vi "report generation.vi"(9 "text":string, 11 "template (empty)":path) -> ()   [LabVIEW 2026]
uses:
  <vilib>/addons/_office/NI_ReportGenerationToolkit.lvlib
  <vilib>/addons/_office/_exclsub.llb/font.ctl
  <vilib>/Utility/NIReport.llb/NI_report.lvclass
  <vilib>/addons/_office/word.llb/Word Easy Table (num).vi
  <vilib>/Utility/NIReport.llb/Report Type.ctl
  <vilib>/Utility/NIReport.llb/NI_ReportGenerationCore.lvlib
panel:
  in  "report type":T1
  in  "error in (no error)":errorcluster
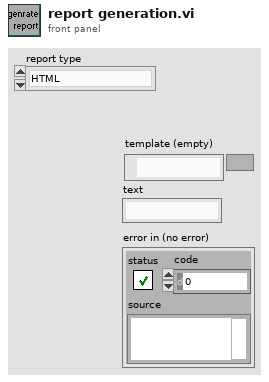
[diagram p1: front panel]
types:
  T1 = typedef "NI_ReportGenerationCore.lvlib/Report Type.ctl" = enum16{"HTML", "Word", "Excel"}
  T2 = typedef "NI_ReportGenerationToolkit.lvlib/font.ctl" = cluster{"font name":string, "font size":dbl, "bold":u16, "italic":u16, "underline":u16, "strike through":u16, "font color":u32}
  T3 = enum16{"maximized", "minimized", "normal", "no change"}
  T4 = enum16{"open", "replace", "create", "open or create", "replace or create", "replace or create with confirmation"}
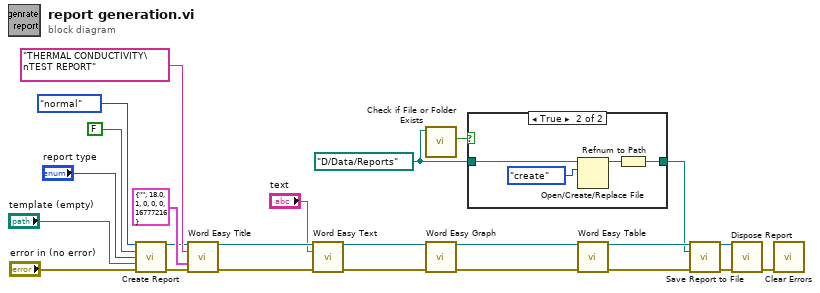
[diagram p0: block diagram]
diagram:
  w8 = path "D:/Data/Reports" ("report file path")
  n1 = call <vilib>:"Create Report.vi"("window state (normal)"=T3."normal", "display alerts? (F)"=FALSE, "report type"="report type", "template (empty)"="template (empty)", "error in (no error)"="error in (no error)") -> ("report out"=w4:refnum<class "NI_report.lvclass">, "error out"=w5:errorcluster)  [unwired: 9 in]
  n2 = call <vilib>:"Word Easy Title.vi"("report in"=w4, "title"="THERMAL CONDUCTIVITY\nTEST REPORT", "font"=T2 {"font name"="", "font size"=18.0, "bold"=1, "italic"=0, "underline"=0, "strike through"=0, "font color"=16777216}, "error in (no error)"=w5) -> ("report out"=w24:refnum<class "NI_report.lvclass">, "error out"=w23:errorcluster)  [unwired: 9 in, 1 out]
  n3 = call <vilib>:"Word Easy Text.vi"("report in"=w24, "text"="text", "error in (no error)"=w23) -> ("report out"=w22:refnum<class "NI_report.lvclass">, "error out"=w21:errorcluster)  [unwired: 10 in, 1 out]
  n4 = call <vilib>:"Check if File or Folder Exists.vi"("path"=w8) -> ("file or folder exists?"=w9:bool)  [unwired: 8 in, 2 out]
  n5 = call <vilib>:"Word Easy Graph.vi"("report in"=w22, "error in (no error)"=w21) -> ("report out"=w20:refnum<class "NI_report.lvclass">, "error out"=w19:errorcluster)  [unwired: 12 in]
  n6 = case shown="True" w9 {
    tunnel: w8 -> [w25 w28]
    tunnel: [w25 w26] -> w10
    frame False {
    }
    frame True {
      n7 = Open/Create/Replace File(file path (use dialog)=w28, operation (0:open)=T4."create") -> (refnum out=w27:refnum<file>)  [unwired: 4 in, 2 out]
      n8 = Refnum to Path(1:w27) -> (0:w26:path)
    }
  }
  n9 = call-poly <vilib>:"Word Easy Table.vi"("report in"=w20, "error in (no error)"=w19) -> ("report out"=w18:refnum<class "NI_report.lvclass">, "error out"=w17:errorcluster)  [unwired: 11 in, 1 out]
  n10 = call-dynamic "Save Report to File.vi"("report in"=w18, "report file path"=w10, "error in (no error)"=w17) -> ("report out"=w15:refnum<class "NI_report.lvclass">, "error out"=w16:errorcluster)  [unwired: 11 in]
  n11 = call-dynamic "Dispose Report.vi"("report in"=w15, "error in (no error)"=w16) -> ("error out"=w14:errorcluster)  [unwired: 13 in]
  n12 = call <vilib>:"Clear Errors.vi"("error in (no error)"=w14) -> ()  [unwired: 5 in, 2 out]
